vi "PicoScope2000aExampleStreamingMSO.vi"() -> ()   [LabVIEW 2010]
doc: "This example demonstrates how to use the PicoScope Labview library to stream data from a PicoScope 2000 Series Device"
uses:
  <vilib>/Waveform/DWDTOps.llb/DWDT Analog to Digital.vi
  PicoScope2000aLib/PicoScope2000aAnalogChannelSettings.ctl
  PicoScope2000aLib/PicoScope2000aDigitalChannelSettings.ctl
panel:
  in  "Port 0 Settings":T1={"Enabled"=FALSE, "Logic Level"=9830} {"Logic Level" items=["1.5V TTL"=9830, "2.5V CMOS"=16383]}
  in  "Channel A Settings":T2={"Enabled"=TRUE, "Coupling"=1, "Range"=6, "Analogue Offset"=0.0} {"Analogue Offset" format="%#_6p"; "Range" items=["20 mV"=1, "50 mV"=2, "100 mV"=3, "200 mV"=4, "500 mV"=5, "1 V"=6, "2 V"=7, "5 V"=8, "10 V"=9, "20 V"=10]; "Coupling" items=["AC", "DC"]}
  out "Analog Channels":T3(graph)
  out "Raw Sample Interval (sec)":dbl=1.0000000130088963e-06 format="%#.5p"
  out "Max ADC value":i16
  out "Chunk time":u32
  out "Elapsed time":dbl
  in  "Poll time (ms)":u32=10 min=1 max=1000 step=1
  in  "Data file":path=path "PicoScope2000aExampleStreaming ChA Data"
  out "size(s)":i32
  out "Queue depth":i32(graph)
  out "queue depth":i32
  in  "Buffer and Transfer Settings":T4={"startIndex"=0, "Samples"=1000000, "Down Sample Ratio"=1, "Down-Sample Mode"=0} {"Down-Sample Mode" items=["None"=0, "Aggregate"=1, "Decimate"=2, "Average"=4]; "Down Sample Ratio" step=1; "Samples" format="%_6p"}
  out "TriggeredAt (In Buffer)":u32 format="%#.6p"
  out "TriggeredAt (Total samples)":u32 format="%#.6p"
  in  "Acquisition Settings":T5={"Auto Stop"=TRUE, "Desired Sample Interval"=1, "Pre-trigger Samples"=0, "Post-trigger Samples"=1000000, "Down-Sample Ratio"=1, "Down-Sample Mode"=0, "Time Units"=3} {"Time Units" items=["Nanoseconds (ns)"=2, "Microseconds (us)"=3, "Milliseconds (ms)"=4, "Seconds (s)"=5]; "Down-Sample Mode" items=["None"=0, "Aggregate"=1, "Decimate"=2, "Average"=4]; "Post-trigger Samples" format="%#.6p"; "Pre-trigger Samples" format="%#_6p"}
  out "Port 0":digitalwaveform(graph)={"t0"=timestamp(0 s since 1904-01-01), "dt"=1.0000000130088963e-06, "Y"={"transitions"=[], "data"=[]}}
  in  "Trigger Settings":T6={"Trigger Enabled"=FALSE, "Trigger Source"=enum."Channel A", "Trigger Threshold (volts)"=0.0, "Trigger Direction"=2, "Trigger Delay (samples)"=0, "Auto Trigger Time (ms)"=1000} {"Trigger Direction" items=["Rising"=2, "Falling"=3]}
  out "Triggered":bool
  out "DownSample Interval (sec)":dbl=1.0000000130088963e-06 format="%#.5p"
  out "Total Samples":u32 format="%#.6p"
  out "Auto Stopped":bool
  in  "Serial Number":string
  in  "Open Using Serial Number":bool
  out "Number of Samples per Capture":u32 format="%#.6p"
  in  "Apply  Settings":bool
  in  "stop":bool
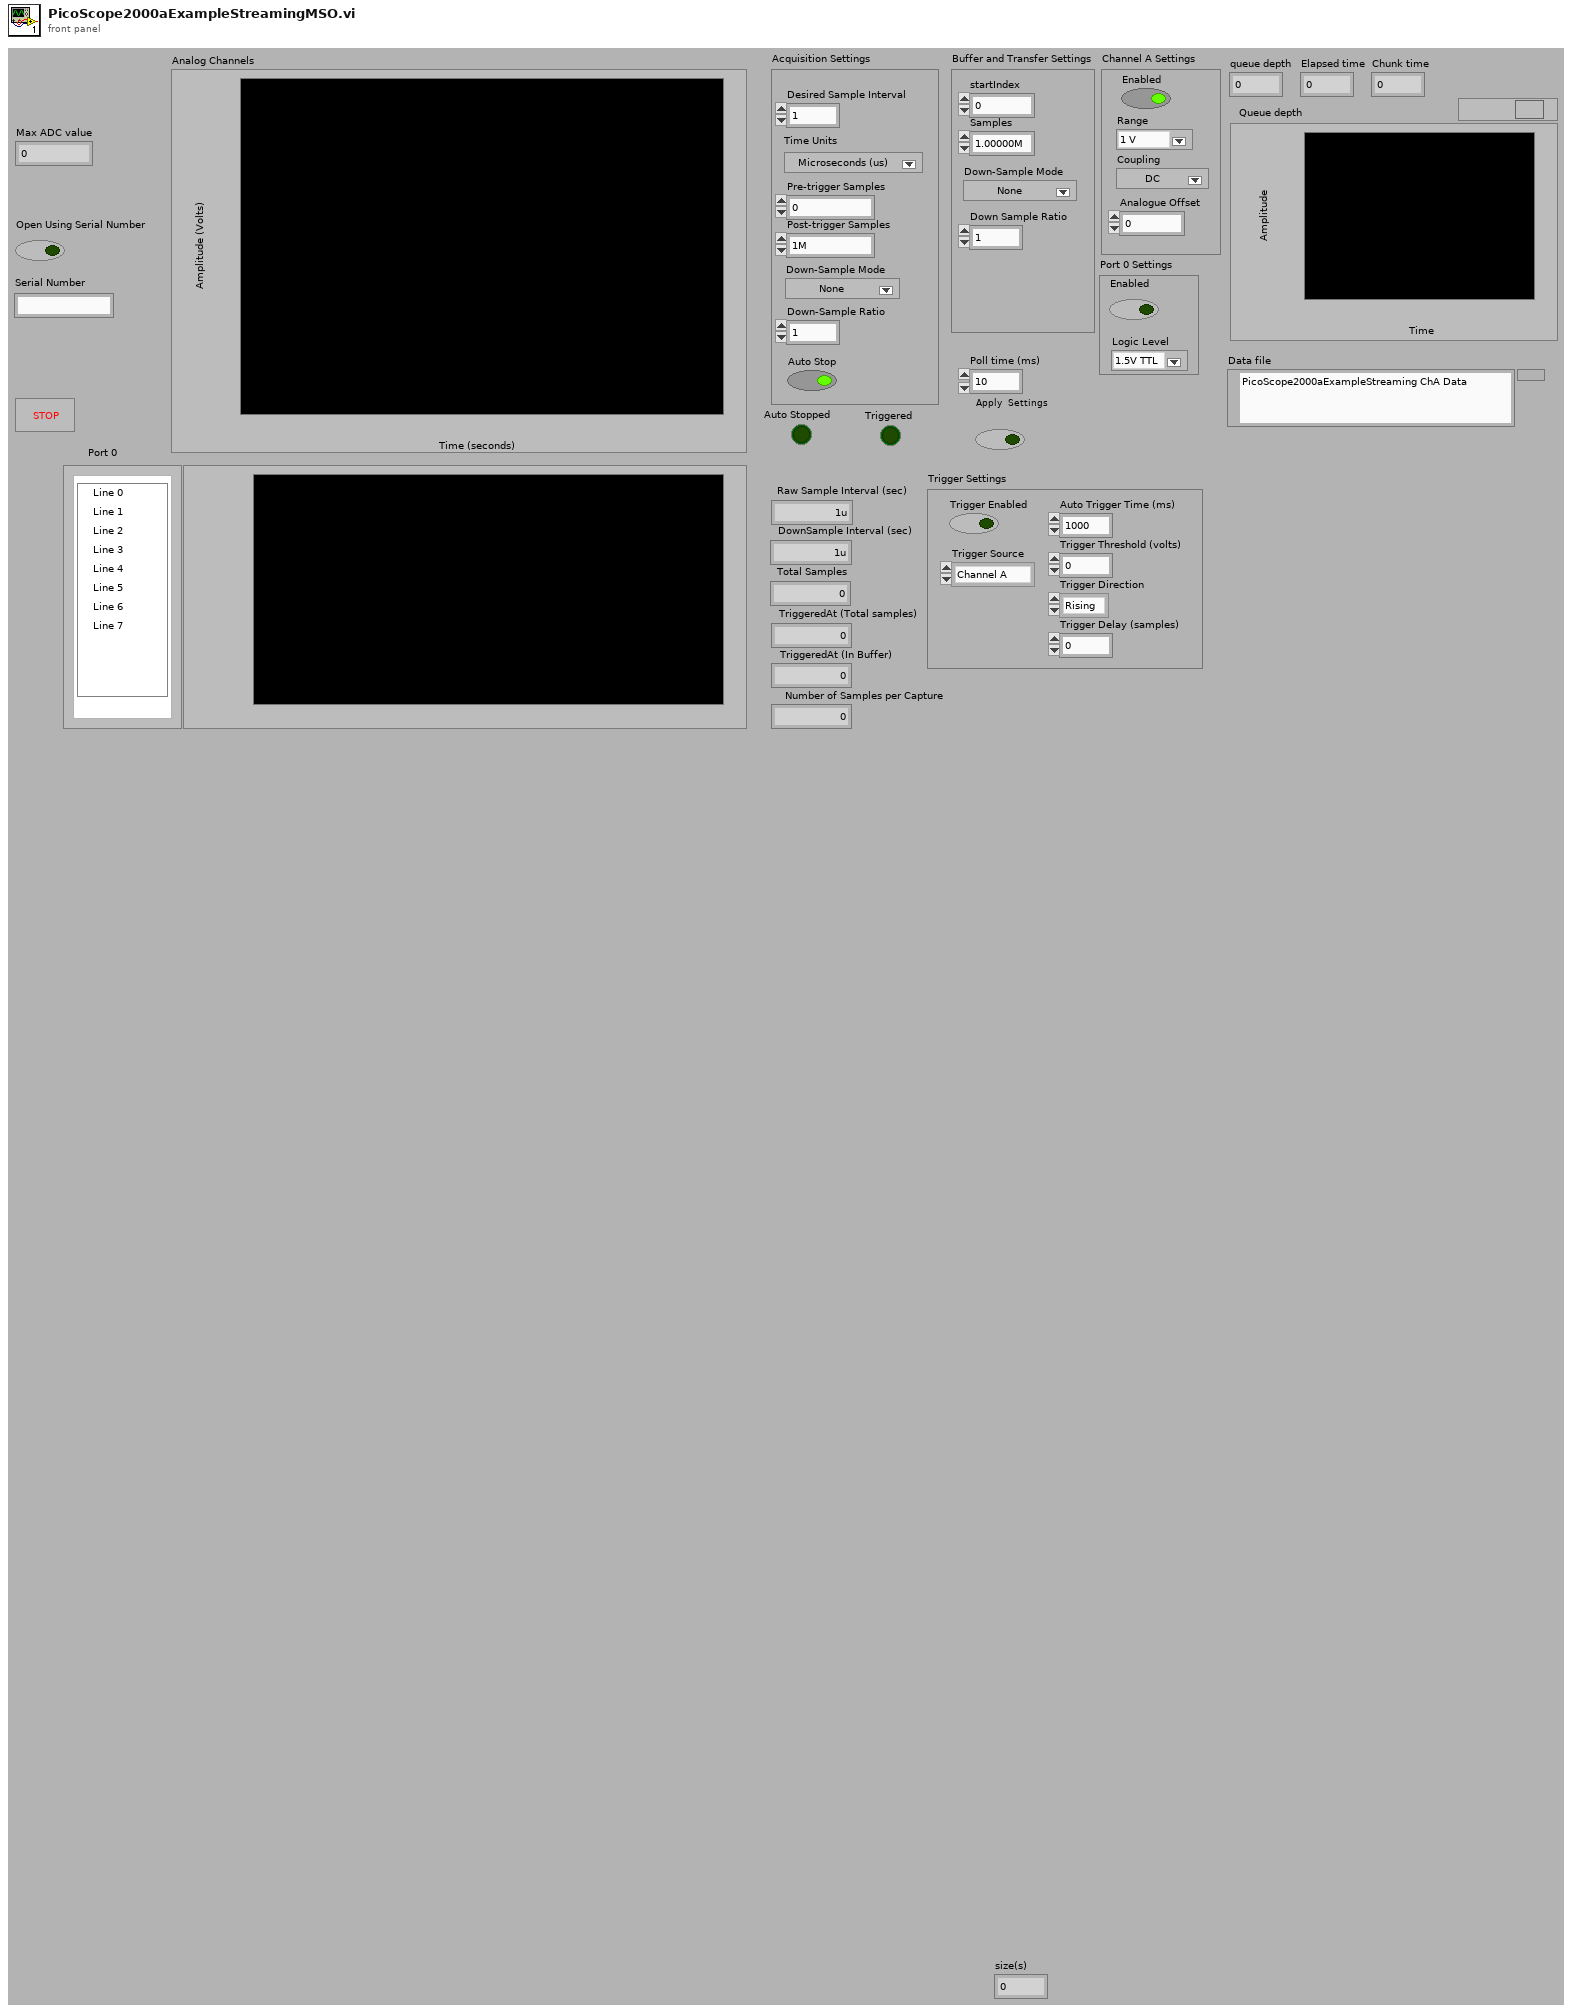
[diagram p1: front panel]
types:
  T1 = typedef "PicoScope2000aDigitalChannelSettings.ctl" = cluster{"Enabled":bool, "Logic Level":i16}
  T2 = typedef "PicoScope2000aAnalogChannelSettings.ctl" = cluster{"Enabled":bool, "Coupling":i16, "Range":u16, "Analogue Offset":sgl}
  T3 = cluster{i32, "DownSample Interval (sec)":dbl, "Data":dbl[]}
  T4 = cluster{"startIndex":u64, "Samples":u64, "Down Sample Ratio":u64, "Down-Sample Mode":u32}
  T5 = cluster{"Auto Stop":bool, "Desired Sample Interval":u32, "Pre-trigger Samples":u32, "Post-trigger Samples":u32, "Down-Sample Ratio":u32, "Down-Sample Mode":i32, "Time Units":u32}
  T6 = cluster{"Trigger Enabled":bool, "Trigger Source":enum16{"Channel A", "Channel B", "Channel C", "Channel D", "Ext."}, "Trigger Threshold (volts)":dbl, "Trigger Direction":u16, "Trigger Delay (samples)":u32, "Auto Trigger Time (ms)":i16}
  T7 = enum16{"open", "open or create", "create or replace", "create", "open (read-only)"}
  T8 = cluster{"Driver Version":string, "USB Version":string, "Hardware":string, "Variant":string, "Batch and Serial":string, "Cal Date":string, "Kernel Version":string, "Digital HW Version":string, "Analogue HW Version":string, "Firmware 1":string, "Firmware 2":string, "MSO":bool, "Number of Channels":i16}
  T9 = cluster{"Channel A Buffer":i16[], "Channel B Buffer":i16[], "Channel C Buffer":i16[], "Channel D Buffer":i16[], "Channel E Buffer":i16[], "Channel F Buffer":i16[], "Channel G Buffer":i16[], "Channel H Buffer":i16[], "Port 0":i16[], "Port 1":i16[]}
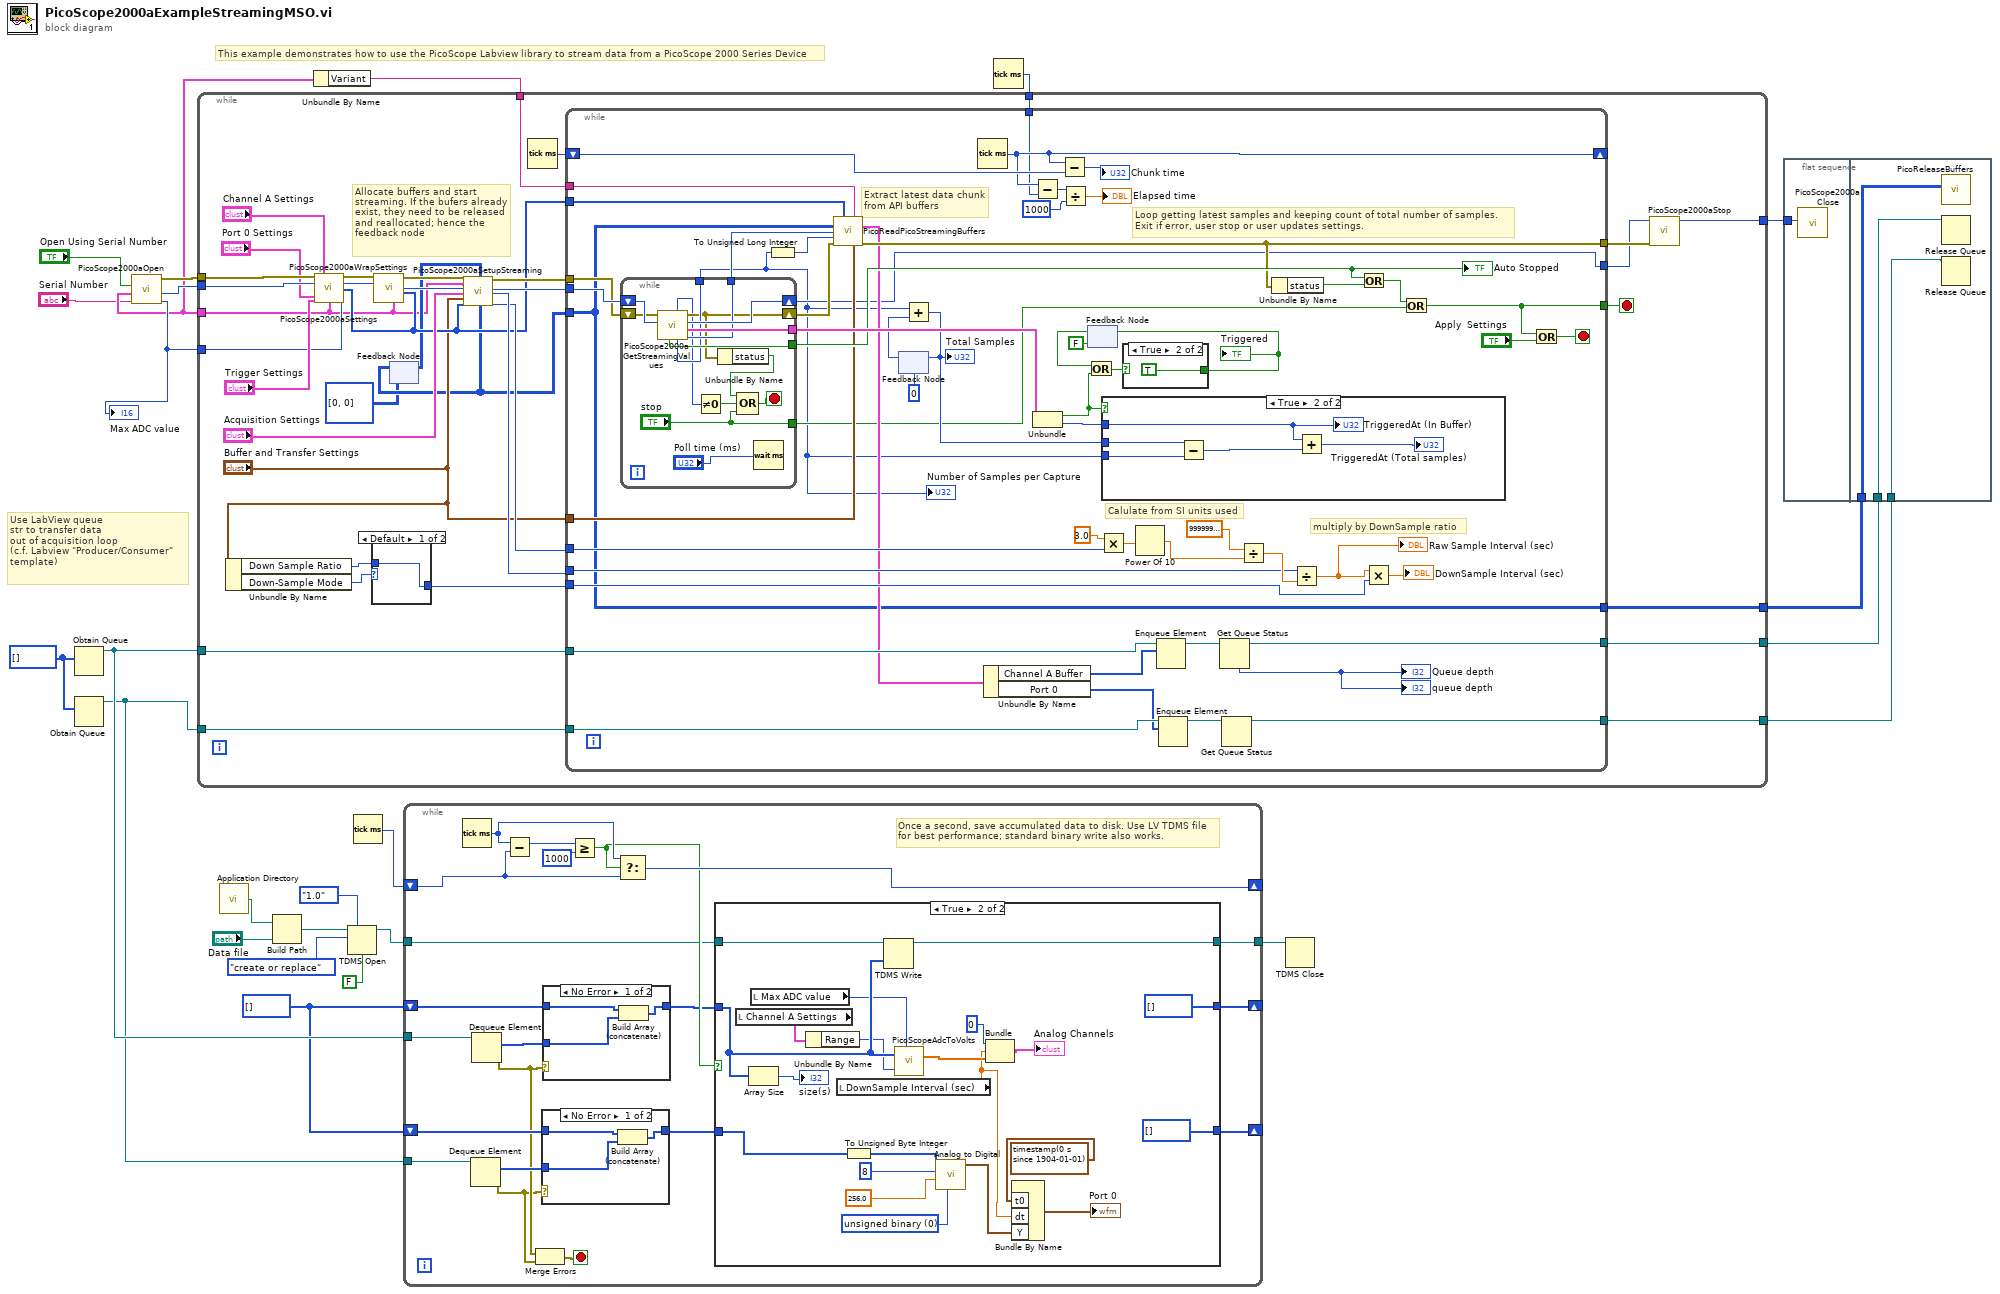
[diagram p0: block diagram]
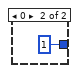
[diagram p5: hidden frame]
diagram:
  w8 = i16[] [] ("History Data")
  w11 = i16[] [] ("History Data")
  # "Use LabView queue\nstr to transfer data\nout of acquisition loop\n(c.f. Labview \"Producer/Consumer\"\ntemplate)"
  # "This example demonstrates how to use the PicoScope Labview library to stream data from a PicoScope 2000 Series Device"
  n1 = Obtain Queue(element data type=w11) -> (queue out=w22:refnum<queue>)  [unwired: 4 in, 2 out]
  n2 = Obtain Queue(element data type=w11) -> (queue out=w9:refnum<queue>)  [unwired: 4 in, 2 out]
  n3 = call "PicoScope2000aOpen.vi"("Serial Number"="Serial Number", "Use Serial Number"="Open Using Serial Number") -> ("Max Adc value"=w23:i16, "handle"=w24:i16, "error out"=w25:errorcluster, "Device Info"=w3:T8)  [unwired: 2 in]
  "Max ADC value" <- w23
  n4 = call <vilib>:"Application Directory.vi"() -> ("Application Directory"=w5:path)
  n5 = Build Path(base path=w5, name or relative path="Data file") -> (appended path=w6:path)
  n6 = Unbundle By Name(w3) -> ("Variant"=w4:string)
  n7 = TDMS Open(6:FALSE ("disable buffering? (T)"), 7:enum16{"1.0", "2.0"}."1.0" ("file format version (2.0)"), 10:T7."create or replace" ("operation (0:open)"), 11:w6) -> (3:w15:refnum<k34>)  [unwired: 2 in, 1 out]
  n8 = Tick Count (ms)() -> (millisecond timer value=w17:u32)
  n9 = while {
    tunnel: w22 -> [w45]
    shift-right: [w36] -> _
    shift-left: w8 -> [w44]
    shift-right: [w39] -> _
    shift-left: w17 -> [w40]
    tunnel: w15 -> [w35]
    tunnel: [w34] -> w14
    tunnel: w9 -> [w32]
    shift-right: [w29] -> _
    shift-left: w8 -> [w31]
    stop <- w28 stop-if-true
    # "Once a second, save accumulated data to disk. Use LV TDMS file\nfor best performance; standard binary write also works."
    n10 = Tick Count (ms)() -> (millisecond timer value=w41:u32)
    n11 = Dequeue Element(queue=w32) -> (element=w33:i16[], error out=w26:errorcluster)  [unwired: 2 in, 2 out]
    n12 = Dequeue Element(queue=w45) -> (element=w46:i16[], error out=w27:errorcluster)  [unwired: 2 in, 2 out]
    n13 = Subtract(x=w41, y=w40) -> (x-y=w43:u32)
    n14 = Merge Errors(w27, w26) -> (w28:errorcluster)
    n15 = case shown="No Error" w26 {
      tunnel: w31 -> [w49 w50]
      tunnel: [w48 w50] -> w30
      tunnel: w33 -> [w47 _]
      frame No Error {
        n16 = Build Array (concatenate)(w49, w47) -> (w48:i16[])
      }
      frame Error {
      }
    }
    n17 = case shown="No Error" w27 {
      tunnel: w44 -> [w77 w78]
      tunnel: [w76 w78] -> w37
      tunnel: w46 -> [w75 _]
      frame No Error {
        n18 = Build Array (concatenate)(w77, w75) -> (w76:i16[])
      }
      frame Error {
      }
    }
    n19 = Greater Or Equal?(x=w43, y=u32 1000) -> (x >= y?=w38:bool)
    n20 = Select(t=w41, s=w38, f=w40) -> (s? t:f=w39:u32)
    n21 = case shown="True" w38 {
      tunnel: w37 -> [w53 w70]
      tunnel: [w53 i16[] [] ("History Data")] -> w36
      tunnel: w35 -> [w52 w72]
      tunnel: [w52 w71] -> w34
      tunnel: w30 -> [w51 w57]
      tunnel: [w51 i16[] [] ("History Data")] -> w29
      frame False {
      }
      frame True {
        w63 = u16 0 items=["unsigned binary", "offset binary", "2's complement"] ("data format (offset binary)")
        n22 = local read "Channel A Settings"() -> (w54:T2)
        n23 = Array Size(array=w70) -> (size(s)=→"size(s)":i32)
        n24 = local read "Max ADC value"() -> (w66:i16)
        n25 = Unbundle By Name(w54) -> ("Range"=w69:u16)
        n26 = local read "DownSample Interval (sec)"() -> (w58:dbl)
        n27 = To Unsigned Byte Integer(number=w57) -> (unsigned 8bit integer=w62:u8[])
        n28 = TDMS Write(0:w72, 9:w70) -> (4:w71:refnum<k34>)  [unwired: 4 in, 3 out]
        n29 = call "PicoScopeAdcToVolts.vi"("Max_adc"=w66, "Range Index"=w69, "Data"=w70) -> ("Data"=w67:dbl[])
        n30 = call-poly <vilib>:"Analog to Digital.vi"("data format (offset binary)"=w63, "full-scale range (pk-pk)"=256.0, "resolution (16 bit)"=8, "analog waveform"=w62) -> ("digital waveform"=w59:digitalwaveform)  [unwired: 4 in, 3 out]
        n31 = Bundle(0, "DownSample Interval (sec)"=w58, "Data"=w67) -> (→"Analog Channels":T3)  [unwired: 1 in]
        n32 = Bundle By Name("t0"=timestamp(0 s since 1904-01-01), "dt"=w58, "Y"=w59) -> (→"Port 0":digitalwaveform)  [unwired: 1 in]
      }
    }
  }
  n33 = Tick Count (ms)() -> (millisecond timer value=w21:u32)
  n34 = while {
    tunnel: [w80] -> w20
    tunnel: w25 -> [w112]
    tunnel: w24 -> [w113]
    tunnel: w3 -> [w82]
    tunnel: w23 -> [w102]
    tunnel: [w95] -> w18
    tunnel: w22 -> [w94]
    tunnel: [w93] -> w19
    tunnel: w21 -> [w90]
    tunnel: [w87] -> w10
    tunnel: w9 -> [w86]
    tunnel: w4 -> [w85]
    stop <- w114 stop-if-true
    # "Allocate buffers and start\nstreaming. If the bufers already\nexist, they need to be released\nand reallocated; hence the\nfeedback node"
    n35 = Unbundle By Name("Buffer and Transfer Settings") -> ("Down Sample Ratio"=w99:u64, "Down-Sample Mode"=w101:u32)
    n36 = call "PicoScope2000aSettings.vi"("error in"=w112, "Channel A Settings"="Channel A Settings", "handle in"=w113, "Trigger Settings"="Trigger Settings", "Port 0 Settings"="Port 0 Settings", "Device Info"=w82, "Max_adc"=w102) -> ("error out"=w107:errorcluster, "handle out"=w106:i16, "Enabled Array"=w97:i16[])  [unwired: 6 in]
    n37 = case shown="Default" w101 {
      tunnel: [w115 u32 1 ("Down-Sample Ratio")] -> w100
      tunnel: w99 -> [w115 _]
      frame Default {
      }
      frame 0 {
      }
    }
    n38 = call "PicoScope2000aWrapSettings.vi"("Device Info"=w82, "Enabled array"=w97, "Handle In"=w106, "error in (no error)"=w107) -> ("Handle Out"=w109:i16, "error out"=w108:errorcluster)  [unwired: 6 in]
    n39 = feedback #1(u64[][] [[0], [0]] ("Pointer array")) -> (w92:u64[][])
    n40 = call "PicoScope2000aSetupStreaming.vi"("error in"=w108, "Device Info"=w82, "handle in"=w109, "Acquisition Settings"="Acquisition Settings", "Buffer and Transfer Settings"="Buffer and Transfer Settings", "enabled array"=w97, "Pointers In"=w92) -> ("Pointer array"=w89:u64[][], "error out"=w110:errorcluster, "handle out"=w111:i16, "Sample Interval"=w104:u32, "sampleIntervalTimeUnits"=w103:u32)  [unwired: 8 in]
    n41 = feedback-in #1(w89) -> ()
    n42 = Tick Count (ms)() -> (millisecond timer value=w91:u32)
    n43 = while {
      tunnel: [w128] -> w79
      tunnel: [w171] -> w114
      tunnel: w111 -> [w147]
      tunnel: w110 -> [w146]
      tunnel: w104 -> [w150]
      tunnel: w103 -> [w158]
      tunnel: [w143] -> w81
      tunnel: w100 -> [w148]
      tunnel: "Buffer and Transfer Settings" -> [w145]
      tunnel: w97 -> [w142]
      tunnel: [w140] -> w95
      tunnel: w94 -> [w138]
      tunnel: w89 -> [w136]
      tunnel: [w136] -> w93
      shift-right: [w131] -> _
      shift-left: w91 -> [w132]
      tunnel: w90 -> [w130]
      tunnel: w85 -> [w125]
      tunnel: [w122] -> w87
      tunnel: w86 -> [w121]
      stop <- w170 stop-if-true
      # "Loop getting latest samples and keeping count of total number of samples. \nExit if error, user stop or user updates settings."
      # "Extract latest data chunk\nfrom API buffers"
      # "Calulate from SI units used"
      # "multiply by DownSample ratio"
      n44 = while {
        tunnel: [w186] -> w169
        tunnel: [w185] -> w166
        tunnel: [w181] -> w126
        tunnel: [w180] -> w117
        shift-right: [w182] -> w128
        shift-left: w147 -> [w184]
        shift-right: [w179] -> w144
        shift-left: w146 -> [w183]
        tunnel: ["stop"] -> w119
        stop <- w174 stop-if-true
        n45 = call "PicoScope2000aGetStreamingValues.vi"("handle in"=w184, "error in"=w183) -> ("Start Index"=w181:u32, "Trigger"=w186:cluster{bool, "triggeredAt":u32}, "handle out"=w182:i16, "error out"=w179:errorcluster, "Number of Samples"=w180:i32, "ready"=w177:i16, "Auto Stopped"=w185:bool)  [unwired: 3 in]
        n46 = Not Equal To 0?(x=w177) -> (x != 0?=w175:bool)
        n47 = Unbundle By Name(w179) -> ("status"=w176:bool)
        n48 = Compound Arithmetic op=OR(w176, w175, "stop") -> (w174:bool)
        n49 = Wait (ms)(milliseconds to wait="Poll time (ms)") -> ()  [unwired: 1 out]
      }
      "Number of Samples per Capture" <- w117
      "Auto Stopped" <- w166
      n50 = To Unsigned Long Integer(number=w117) -> (unsigned 32bit integer=w118:u32)
      n51 = call "PicoReadPicoStreamingBuffers.vi"("enabled array"=w142, "Buffer and Transfer Settings"=w145, "Variant"=w125, "Pointer array"=w136, "Offset Index"=w126, "Number of Samples"=w118, "error in (no error)"=w144) -> ("Buffers (Max or non-aggregated)"=w137:T9, "error out"=w143:errorcluster)  [unwired: 6 in, 1 out]
      n52 = feedback #2(u32 0) -> (w162:u32)
      n53 = Add(x=w117, y=w162) -> (x+y=w154:u32)
      "Total Samples" <- w154
      n54 = feedback-in #2(w154) -> ()
      n55 = Tick Count (ms)() -> (millisecond timer value=w131:u32)
      n56 = Unbundle By Name(w137) -> ("Channel A Buffer"=w127:i16[], "Port 0"=w120:i16[])
      n57 = Subtract(x=w131, y=w130) -> (x-y=w135:u32)
      n58 = Unbundle(w169) -> (w152:bool, "triggeredAt"=w151:u32)
      n59 = Subtract(x=w131, y=w132) -> (x-y=→"Chunk time":u32)
      n60 = Divide(x=w135, y=u32 1000) -> (x/y=→"Elapsed time":dbl)
      n61 = feedback #3(FALSE) -> (w164:bool)
      n62 = Or(x=w164, y=w152) -> (x .or. y?=w155:bool)
      n63 = Multiply(x=3.0, y=w158) -> (x*y=w156:dbl)
      n64 = case shown="True" w152 {
        tunnel: w117 -> [_ w187]
        tunnel: w154 -> [_ w191]
        tunnel: w151 -> [_ w189]
        frame False {
        }
        frame True {
          n65 = Subtract(x=w191, y=w187) -> (x-y=w190:u32)
          n66 = Add(x=w189, y=w190) -> (x+y=→"TriggeredAt (Total samples)":u32)
          "TriggeredAt (In Buffer)" <- w189
        }
      }
      n67 = case shown="True" w155 {
        selector: w155 -> [w192 _]
        tunnel: [w192 TRUE] -> w153
        frame False {
        }
        frame True {
        }
      }
      "Triggered" <- w153
      n68 = feedback-in #3(w153) -> ()
      n69 = Power Of 10(x=w156) -> (10^x=w157:dbl)
      n70 = Enqueue Element(queue=w138, element=w127) -> (queue out=w139:refnum<queue>)  [unwired: 2 in, 2 out]
      n71 = Enqueue Element(queue=w121, element=w120) -> (queue out=w123:refnum<queue>)  [unwired: 2 in, 2 out]
      n72 = Get Queue Status(queue=w139) -> (queue out=w140:refnum<queue>, # elements in queue=→"queue depth" →"Queue depth":i32)  [unwired: 2 in, 6 out]
      n73 = Get Queue Status(queue=w123) -> (queue out=w122:refnum<queue>)  [unwired: 2 in, 7 out]
      n74 = Divide(x=sgl 1000000000000000.0 ("y"), y=w157) -> (x/y=w159:dbl)
      n75 = Unbundle By Name(w143) -> ("status"=w168:bool)
      n76 = Divide(x=w150, y=w159) -> (x/y=w124:dbl)
      "Raw Sample Interval (sec)" <- w124
      n77 = Or(x=w166, y=w168) -> (x .or. y?=w167:bool)
      n78 = Multiply(x=w124, y=w148) -> (x*y=→"DownSample Interval (sec)":dbl)
      n79 = Or(x=w167, y=w119) -> (x .or. y?=w171:bool)
      n80 = Or(x=w171, y="Apply  Settings") -> (x .or. y?=w170:bool)
    }
    n81 = call "PicoScope2000aStop.vi"("error in (no error)"=w81, "handle in"=w79) -> ("handle out"=w80:i16)  [unwired: 8 in, 1 out]
  }
  n82 = TDMS Close(11:w14) -> ()  [unwired: 1 in, 2 out]
  n83 = flat-sequence {
    tunnel: w20 -> [w194]
    tunnel: w19 -> [w197]
    tunnel: w18 -> [w196]
    tunnel: w10 -> [w195]
    frame #0 {
      n84 = call "PicoScope2000aClose.vi"("handle"=w194) -> ()
    }
    frame #1 {
      n85 = call "PicoReleaseBuffers.vi"("Pointer array"=w197) -> ()  [unwired: 10 in, 1 out]
      n86 = Release Queue(queue=w196) -> ()  [unwired: 2 in, 3 out]
      n87 = Release Queue(queue=w195) -> ()  [unwired: 2 in, 3 out]
    }
  }
